vi "Parse Rig IO List.vi"(8 "error in":errorcluster, 11 "JSON string":string) -> (0 "error out":errorcluster, 3 "IO List":cluster{"name":string, "type":string}[](array[cluster]))   [LabVIEW 2026]
doc: "Reads the name and type of every channel from a rig JSON document. AF-free."
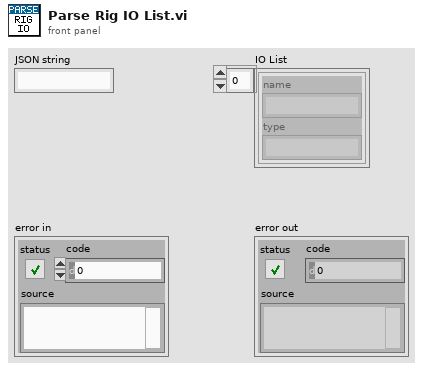
[diagram p1: front panel]
types:
  T1 = cluster{"channels":cluster{"name":string, "type":string}[]}
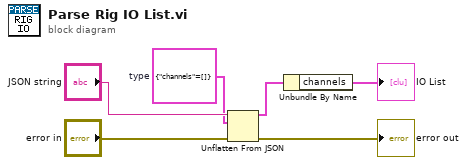
[diagram p0: block diagram]
diagram:
  w5 = T1 {"channels"=[]}  # type
  n1 = Unflatten From JSON(JSON string="JSON string", type and defaults=w5, error in (no error)="error in") -> (value=w3:T1, error out=→"error out":errorcluster)  [unwired: 4 in]
  n2 = Unbundle By Name(w3) -> ("channels"=→"IO List":cluster{"name":string, "type":string}[])
